vi "Template Message Path.vi"() -> (2 "Template Library Path":path)   [LabVIEW 2020, in "LV-Protoc.lvlib"]
uses:
  LV-Protoc.lvlib
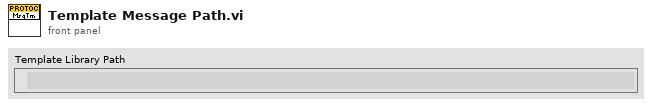
[diagram p1: front panel]
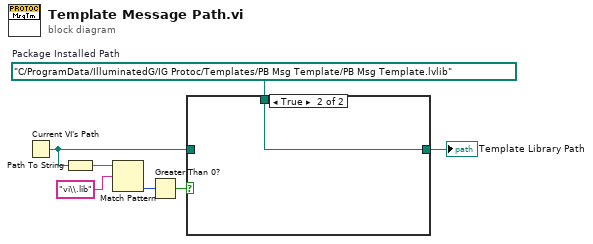
[diagram p0: block diagram]
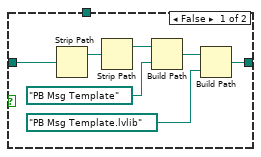
[diagram p2: hidden frame]
diagram:
  w2 = path "C:/ProgramData/IlluminatedG/IG Protoc/Templates/PB Msg Template/PB Msg Template.lvlib"  # Package Installed Path
  n1 = Current VI's Path() -> (path=w4:path)
  n2 = Path To String(path=w4) -> (string=w7:string)
  n3 = Match Pattern(string=w7, regular expression="vi\\.lib") -> (offset past match=w5:i32)  [unwired: 1 in, 3 out]
  n4 = Greater Than 0?(x=w5) -> (x > 0?=w3:bool)
  n5 = case shown="True" w3 {
    tunnel: [w9 w15] -> w1
    tunnel: w4 -> [w8 _]
    tunnel: w2 -> [_ w15]
    frame False {
      n6 = Strip Path(path=w8) -> (stripped path=w14:path)  [unwired: 1 out]
      n7 = Strip Path(path=w14) -> (stripped path=w13:path)  [unwired: 1 out]
      n8 = Build Path(base path=w13, name or relative path=path "PB Msg Template") -> (appended path=w11:path)
      n9 = Build Path(base path=w11, name or relative path=path "PB Msg Template.lvlib") -> (appended path=w9:path)
    }
    frame True {
    }
  }
  "Template Library Path" <- w1
